vi "Get MB Address from Parameter Name.vi"(10 "Key":string, 11 "MB Coils":T1[](array[typedef])) -> (3 "Address":u16)   [LabVIEW 2021]
uses:
  Modbus Address Cluster.ctl
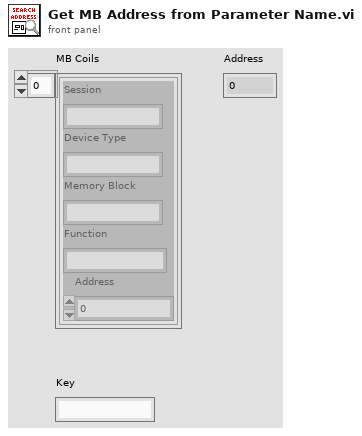
[diagram p1: front panel]
types:
  T1 = typedef "Modbus Address Cluster.ctl" = cluster{"Session":string, "Device Type":string, "Memory Block":string, "Function":string, "Address":u16}
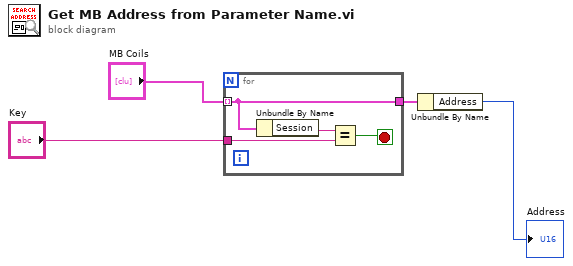
[diagram p0: block diagram]
diagram:
  n1 = for {
    tunnel: "MB Coils" -> [w6] mode=indexing
    tunnel: "Key" -> [w7]
    tunnel: [w6] -> w3
    stop <- w5 stop-if-true
    n2 = Unbundle By Name(w6) -> ("Session"=w8:string)
    n3 = Equal?(x=w8, y=w7) -> (x = y?=w5:bool)
  }
  n4 = Unbundle By Name(w3) -> ("Address"=→"Address":u16)
